vi "Generate code.vi"(1 "Terms":T1[](array[typedef]), 3 "Diagram":refnum<vi>, 5 "XRef":refnum<vi>, 6 "State In":T4) -> (0 "Generated Code?":bool, 2 "State Out":T4, 4 "Reply":string[](array[string]))   [LabVIEW 2012, in "OpenG FilterArray.xnode"]
uses:
  OpenG FilterArray.xnode
  State.ctl
  <vilib>/XNodeSupport/XNodeTermIDPair.ctl
  <vilib>/XNodeSupport/XNodeTermRef.ctl
  <vilib>/XNodeSupport/XNodeString.ctl
  <vilib>/Utility/miscctls.llb/LVPositionTypeDef.ctl
  <userlib>/_LAVAcr/Scripting Tools/Scripting Tools.lvlib
  <vilib>/XNodeSupport/NI_XNodeSupport.lvlib
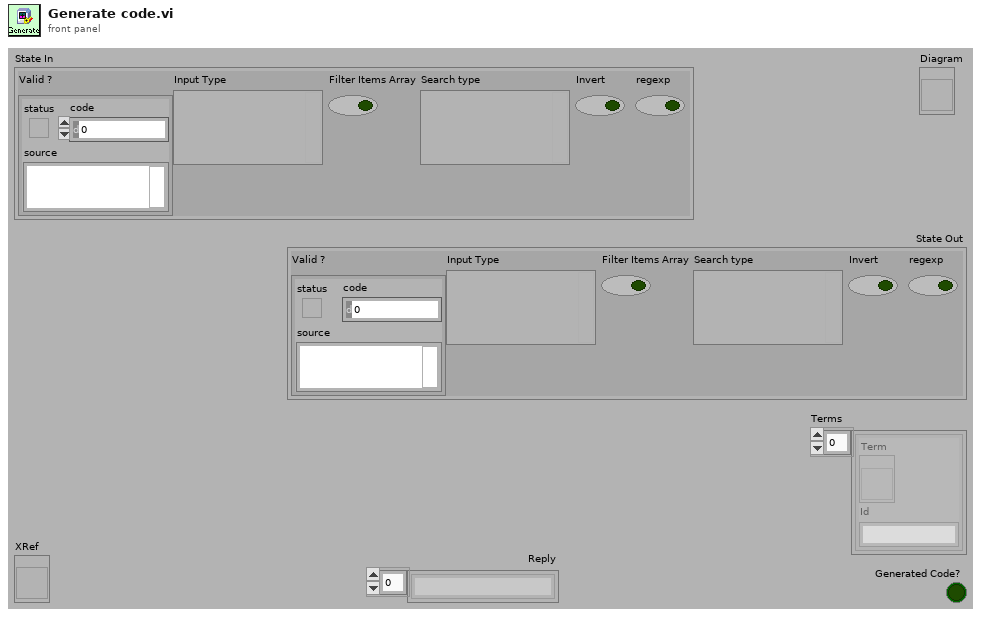
[diagram p1: front panel]
types:
  T1 = typedef "NI_XNodeSupport.lvlib/XNodeTermIDPair.ctl" = cluster{"Term":T2, "Id":T3}
  T2 = typedef "NI_XNodeSupport.lvlib/XNodeTermRef.ctl" = refnum<vi>
  T3 = typedef "NI_XNodeSupport.lvlib/XNodeString.ctl" = string
  T4 = typedef "OpenG FilterArray.xnode/State.ctl" = cluster{"Valid ?":errorcluster, "Input Type":variant, "Filter Items Array":bool, "Search type":variant, "Invert":bool, "regexp":bool}
  T5 = typedef "LVPositionTypeDef.ctl" = cluster{"Left":i32, "Top":i32}
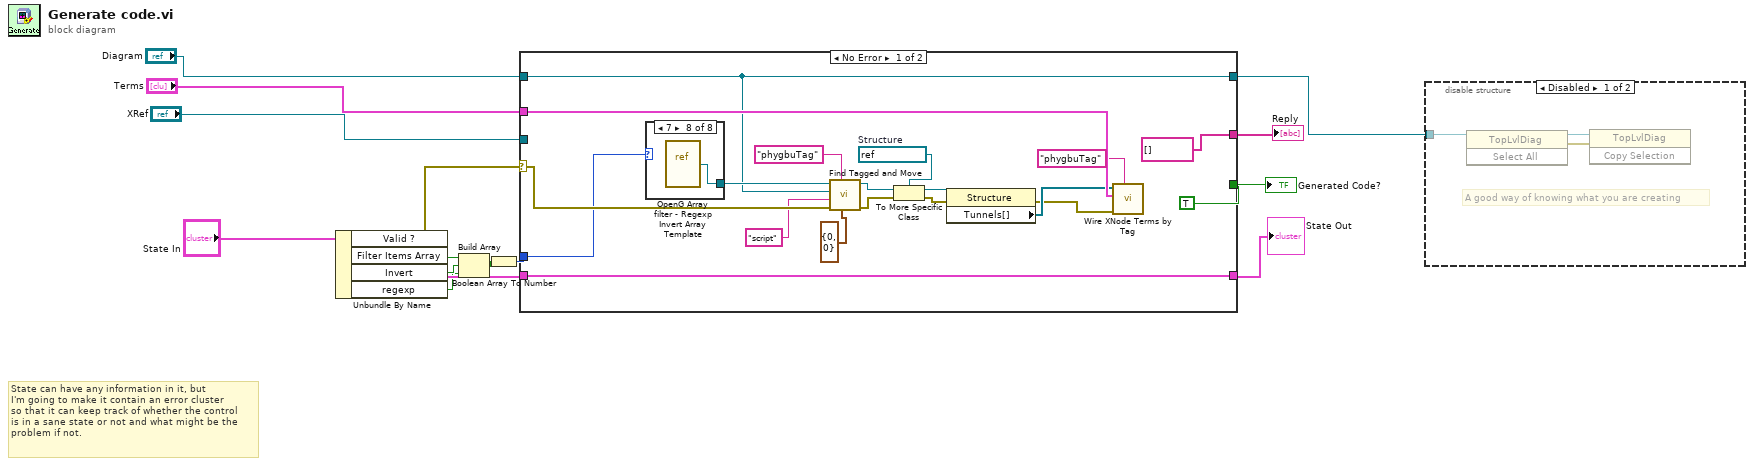
[diagram p0: block diagram]
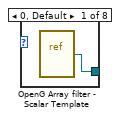
[diagram p2: hidden frame]
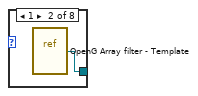
[diagram p3: hidden frame]
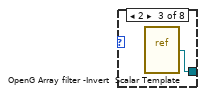
[diagram p4: hidden frame]
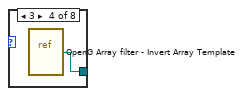
[diagram p5: hidden frame]
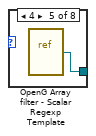
[diagram p6: hidden frame]
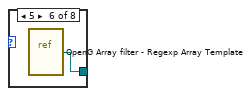
[diagram p7: hidden frame]
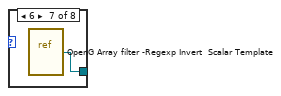
[diagram p8: hidden frame]
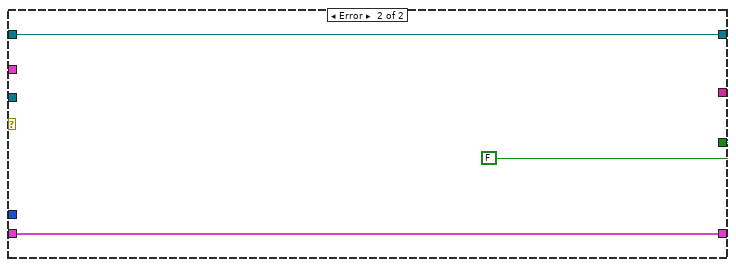
[diagram p9: hidden frame]
diagram:
  # "State can have any information in it, but\nI'm going to make it contain an error cluster\nso that it can keep track of whether the control\nis in a sane state or not and what might be the\nproblem if not."
  n1 = Unbundle By Name("State In") -> ("Valid ?"=w14:errorcluster, "Filter Items Array"=w4:bool, "Invert"=w3:bool, "regexp"=w1:bool)
  n2 = Build Array(w4, w3, w1) -> (w5:bool[])
  n3 = Boolean Array To Number(Boolean array=w5) -> (number=w2:u32)
  n4 = case shown="No Error" w14 {
    selector: w14 -> [w26 _]
    tunnel: "State In" -> [w31 w44]
    tunnel: "Diagram" -> [w24 w42]
    tunnel: "Terms" -> [w30 _]
    tunnel: "XRef" -> [_ _]
    tunnel: [w24 w42] -> w6
    tunnel: [string[] [] ("Reply") _] -> w9
    tunnel: [TRUE FALSE] -> w8
    tunnel: [w31 w44] -> w7
    tunnel: w2 -> [w15 _]
    frame No Error {
      w28 = refnum<vi> refnum  # Structure
      n5 = case shown="7" w15 {
        tunnel: [w34 w35 w36 w37 w38 w39 w40 w41] -> w25
        frame 0, Default {
          n6 = vi-ref "OpenG Array filter - Scalar Template.vi"() -> (w34:refnum<vi>)
        }
        frame 1 {
          n7 = vi-ref "OpenG Array filter - Template.vi"() -> (w35:refnum<vi>)
        }
        frame 2 {
          n8 = vi-ref "OpenG Array filter -Invert  Scalar Template.vi"() -> (w36:refnum<vi>)
        }
        frame 3 {
          n9 = vi-ref "OpenG Array filter - Invert Array Template.vi"() -> (w37:refnum<vi>)
        }
        frame 4 {
          n10 = vi-ref "OpenG Array filter - Scalar Regexp Template.vi"() -> (w38:refnum<vi>)
        }
        frame 5 {
          n11 = vi-ref "OpenG Array filter - Regexp Array Template.vi"() -> (w39:refnum<vi>)
        }
        frame 6 {
          n12 = vi-ref "OpenG Array filter -Regexp Invert  Scalar Template.vi"() -> (w40:refnum<vi>)
        }
        frame 7 {
          n13 = vi-ref "OpenG Array filter - Regexp Invert Array Template.vi"() -> (w41:refnum<vi>)
        }
      }
      n14 = call <userlib>:"Find Tagged and Move.vi"("position"=T5 {"Left"=0, "Top"=0}, "TagName"="phygbuTag", "error in"=w26, "TagValue"="script", "Destination Diagram"=w24, "VI Refnum"=w25) -> ("error out"=w19:errorcluster, "Moved Tagged object"=w20:refnum<vi>)  [unwired: 4 out]
      n15 = To More Specific Class(target class=w28, reference=w20, error in=w19) -> (specific class reference=w29:refnum<vi>, error out=w18:errorcluster)
      n16 = property class="Structure"(reference=w29, error in=w18) -> (error out=w17:errorcluster, "Tunnels[]"=w27:refnum<vi>[])  [unwired: 1 out]
      n17 = call <userlib>:"Wire XNode Terms by Tag.vi"("TagName"="phygbuTag", "error in (no error)"=w17, "Term Refs"=w30, "Source References"=w27) -> ()  [unwired: 8 out]
    }
    frame Error {
    }
  }
  "State Out" <- w7
  "Reply" <- w9
  "Generated Code?" <- w8
  n18 = disable-structure shown="Disabled" {
    disable-tunnel: w6 -> [w45 _]
    frame Disabled {
      # "A good way of knowing what you are creating"
      n19 = invoke class="TopLvlDiag" method="Select All"(reference=w45) -> (reference out=w47:refnum<vi>, error out=w46:errorcluster)  [unwired: 2 in, 1 out]
      n20 = invoke class="TopLvlDiag" method="Copy Selection"(reference=w47, error in=w46) -> ()  [unwired: 1 in, 3 out]
    }
    frame Enabled {
    }
  }
